vi "midiOutClose.vi"(8 "error in":errorcluster, 11 "midi in":refnum<class "midi.lvclass">) -> (0 "error out":errorcluster, 3 "midi out":refnum<class "midi.lvclass">)   [LabVIEW 2020, in "midi.lvclass"]
doc: "The midiOutClose function closes the specified MIDI output device."
uses:
  midi.lvclass
  midi.lvclass/midi.ctl
  winmm.dll
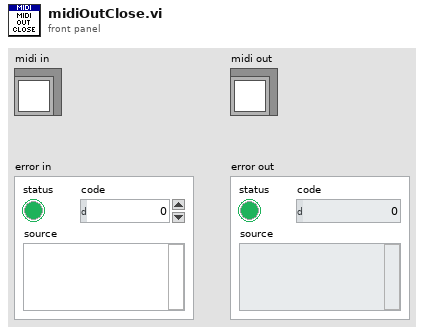
[diagram p1: front panel]
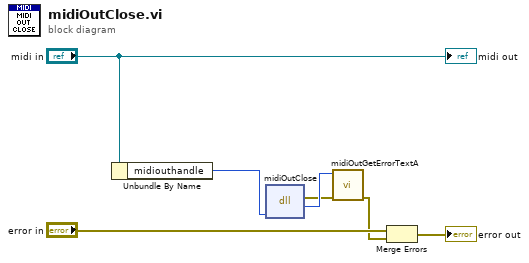
[diagram p0: block diagram]
diagram:
  n1 = Unbundle By Name("midi in") -> ("midiouthandle"=w4:u64)
  n2 = dll-call lib="winmm.dll" fn="midiOutClose"("hmidiout"=w4) -> (error out=w5:errorcluster, "return type"=w7:i32)  [unwired: 4 in, 1 out]
  n3 = call "midiOutGetErrorTextA.vi"("error in"=w5, "Error Code"=w7) -> ("error out"=w2:errorcluster)  [unwired: 9 in]
  n4 = Merge Errors("error in", w2) -> (→"error out":errorcluster)
  "midi out" <- "midi in"
